vi "CSE ISP - RW Control Values to INI file.vi"(6 "cmd (read)":enum16{"read", "write"}(ring), 8 "error in":errorcluster, 10 "Ctrl refnums":refnum<vi>[](array[refnum]), 11 "INI refnum":T1) -> (0 "error out":errorcluster, 3 "dup INI refnum":T1)   [LabVIEW 2021]
doc: "::: CalcExpress Toolkit :::\nCopyright (c) 2000-2026 Konstantin Shifershteyn. All rights reserved."
uses:
  <vilib>/Utility/config.llb/Config Data RefNum.ctl
  <vilib>/Utility/config.llb/Write Key (Path).vi
  <vilib>/Utility/config.llb/Read Key (Path).vi
  <vilib>/Utility/config.llb/NI_LVConfig.lvlib
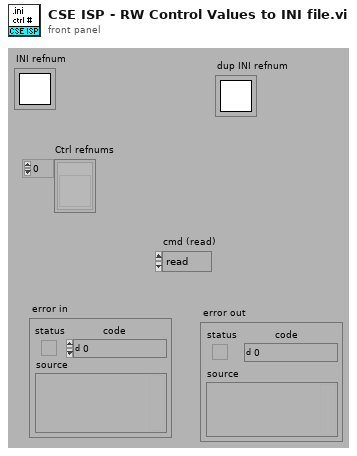
[diagram p1: front panel]
types:
  T1 = typedef "NI_LVConfig.lvlib/Config Data RefNum.ctl" = refnum<k1>
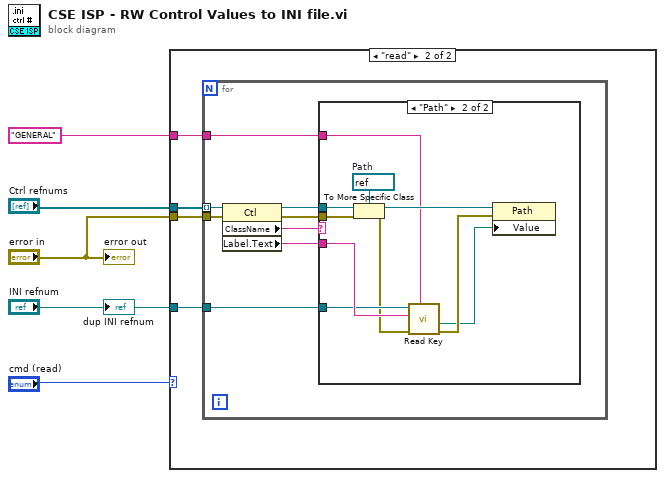
[diagram p0: block diagram]
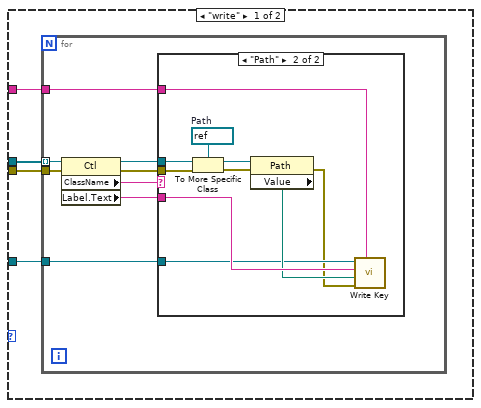
[diagram p2: hidden frame]
diagram:
  n1 = case shown="\"read\"" "cmd (read)" {
    tunnel: "Ctrl refnums" -> [w9 w31]
    tunnel: "error in" -> [w8 w30]
    tunnel: "INI refnum" -> [w7 w29]
    tunnel: "GENERAL" -> [w6 w28]
    frame "write" {
      n2 = for {
        tunnel: w9 -> [w14] mode=indexing
        tunnel: w7 -> [w13]
        tunnel: w8 -> [w11]
        tunnel: w6 -> [w10]
        n3 = property class="Ctl"(reference=w14, error in=w11) -> (reference out=w16:refnum<vi>, error out=w12:errorcluster, "ClassName"=w17:string, "Label.Text"=w15:string)
        n4 = case shown="\"Path\"" w17 {
          tunnel: w16 -> [_ w27]
          tunnel: w15 -> [_ w24]
          tunnel: w13 -> [_ w22]
          tunnel: w12 -> [_ w21]
          tunnel: w10 -> [_ w18]
          frame Default {
          }
          frame "Path" {
            w25 = refnum<vi> refnum  # Path
            n5 = To More Specific Class(target class=w25, reference=w27, error in=w21) -> (specific class reference=w26:refnum<vi>, error out=w20:errorcluster)
            n6 = property class="Path"(reference=w26, error in=w20) -> (error out=w19:errorcluster, "Value"=w23:path)  [unwired: 1 out]
            n7 = call-poly <vilib>:"Write Key.vi"("section"=w18, "error in (no error)"=w19, "value"=w23, "key"=w24, "refnum"=w22) -> ()  [unwired: 4 in, 3 out]
          }
        }
      }
    }
    frame "read" {
      n8 = for {
        tunnel: w31 -> [w36] mode=indexing
        tunnel: w29 -> [w35]
        tunnel: w30 -> [w33]
        tunnel: w28 -> [w32]
        n9 = property class="Ctl"(reference=w36, error in=w33) -> (reference out=w38:refnum<vi>, error out=w34:errorcluster, "ClassName"=w39:string, "Label.Text"=w37:string)
        n10 = case shown="\"Path\"" w39 {
          tunnel: w38 -> [_ w49]
          tunnel: w37 -> [_ w46]
          tunnel: w35 -> [_ w45]
          tunnel: w34 -> [_ w44]
          tunnel: w32 -> [_ w41]
          frame Default {
          }
          frame "Path" {
            w47 = refnum<vi> refnum  # Path
            n11 = To More Specific Class(target class=w47, reference=w49, error in=w44) -> (specific class reference=w48:refnum<vi>, error out=w43:errorcluster)
            n12 = call-poly <vilib>:"Read Key.vi"("section"=w41, "error in (no error)"=w43, "key"=w46, "refnum"=w45) -> ("error out"=w42:errorcluster, "value"=w40:path)  [unwired: 4 in, 2 out]
            n13 = property class="Path"(reference=w48, error in=w42, "Value"=w40) -> ()  [unwired: 2 out]
          }
        }
      }
    }
  }
  "error out" <- "error in"
  "dup INI refnum" <- "INI refnum"
